vi "Start VI.vi"(11 "Command Line Arguments":string[](array[string])) -> (2 "Output":string, 3 "Exit Code":i32)   [LabVIEW 2020]
doc: "Starts another VI in this LabVIEW instance without waiting for it to finish, and returns at once. CI helper for LabVIEW CLI: RunVI only runs VIs with its own connector pane, so an ordinary top-level VI (an example server with a While Loop and a Stop button) is started through this one (LabVIEWCLI -OperationName RunVI -VIPath this VI arg0).\n\nCommand Line Arguments: [0] absolute path of the VI to start; further elements are ignored. The VI is opened with Open VI Reference, refused when its Execution:State is Bad, and otherwise started with Run VI, Wait until done FALSE and Auto Dispose Ref TRUE, so it keeps running after this VI returns and its reference is released when it stops.\n\nExit Code is 0 when the VI was started and 1 otherwise (no path given, file missing, VI broken, any error). Output is a one-line summary. Errors are reported in Output and cleared at the end, so this VI always returns."
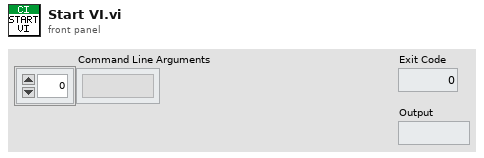
[diagram p1: front panel]
types:
  T1 = enum32{"Bad", "Idle", "Run top level", "Running"}
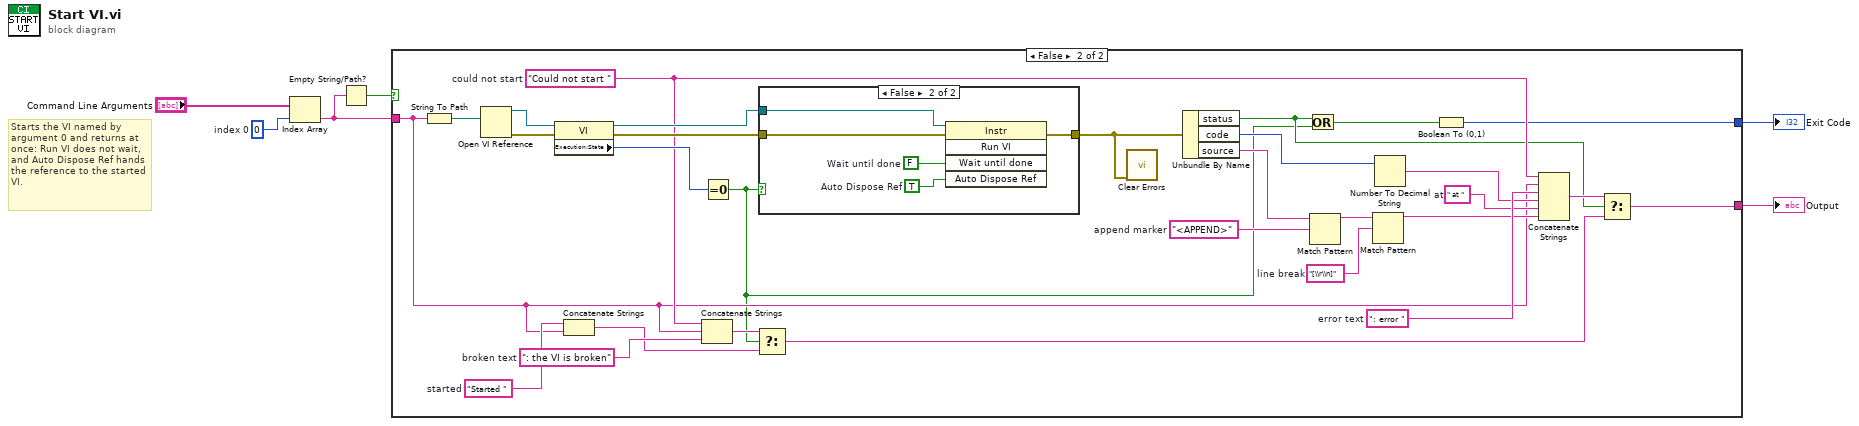
[diagram p0: block diagram]
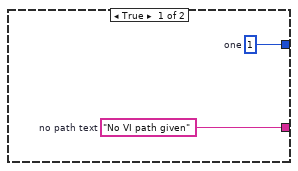
[diagram p2: hidden frame]
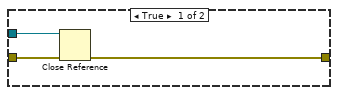
[diagram p3: hidden frame]
diagram:
  w5 = 0  # index 0
  # "Starts the VI named by argument 0 and returns at once: Run VI does not wait, and Auto Dispose Ref hands the reference to the started VI."
  n1 = Index Array(array="Command Line Arguments", index=w5) -> (element=w4:string)
  n2 = Empty String/Path?(string/path=w4) -> (empty?=w3:bool)
  n3 = case shown="False" w3 {
    tunnel: w4 -> [_ w18]
    tunnel: [w8 w10] -> w2
    tunnel: [w7 w9] -> w1
    frame True {
      w7 = "No VI path given"  # no path text
      w8 = 1  # one
    }
    frame False {
      w27 = "[\\r\\n]"  # line break
      w29 = "<APPEND>"  # append marker
      w19 = "Started "  # started
      w20 = ": the VI is broken"  # broken text
      w23 = " at "  # at
      w25 = ": error "  # error text
      w21 = "Could not start "  # could not start
      n4 = String To Path(string=w18) -> (path=w37:path)
      n5 = Open VI Reference(vi path=w37) -> (vi reference=w36:refnum<vi>, error out=w35:errorcluster)  [unwired: 5 in]
      n6 = property class="VI"(reference=w36, error in=w35) -> (reference out=w33:refnum<vi>, error out=w32:errorcluster, "Execution:State"=w34:T1)
      n7 = Concatenate Strings(w19, w18) -> (w16:string)
      n8 = Concatenate Strings(w21, w18, w20) -> (w17:string)
      n9 = Equal To 0?(x=w34) -> (x = 0?=w12:bool)
      n10 = Select(t=w17, s=w12, f=w16) -> (s? t:f=w14:string)
      n11 = case shown="False" w12 {
        tunnel: w33 -> [w40 w45]
        tunnel: w32 -> [w39 w44]
        tunnel: [w38 w41] -> w31
        frame True {
          n12 = Close Reference(reference=w40, error in (no error)=w39) -> (error out=w38:errorcluster)
        }
        frame False {
          w42 = TRUE  # Auto Dispose Ref
          w43 = FALSE  # Wait until done
          n13 = invoke class="Instr" method="Run VI"(reference=w45, error in=w44, "Wait until done"=w43, "Auto Dispose Ref"=w42) -> (error out=w41:errorcluster)  [unwired: 1 in, 4 out]
        }
      }
      n14 = call <vilib>:"Clear Errors.vi"("error in (no error)"=w31) -> ()  [unwired: 5 in, 2 out]
      n15 = Unbundle By Name(w31) -> ("status"=w13:bool, "code"=w26:i32, "source"=w30:string)
      n16 = Or(x=w13, y=w12) -> (x .or. y?=w11:bool)
      n17 = Match Pattern(string=w30, regular expression=w29) -> (before substring=w28:string)  [unwired: 1 in, 3 out]
      n18 = Match Pattern(string=w28, regular expression=w27) -> (before substring=w22:string)  [unwired: 1 in, 3 out]
      n19 = Number To Decimal String(number=w26) -> (decimal integer string=w24:string)  [unwired: 1 in]
      n20 = Boolean To (0,1)(Boolean=w11) -> (0, 1=w10:i16)
      n21 = Concatenate Strings(w21, w18, w25, w24, w23, w22) -> (w15:string)
      n22 = Select(t=w15, s=w13, f=w14) -> (s? t:f=w9:string)
    }
  }
  "Exit Code" <- w2
  "Output" <- w1
